vi "Table_CellValue_Tests.vi"(8 "error in":errorcluster) -> (0 "error out":errorcluster)   [LabVIEW 2016, in "DronaTest.lvlib"]
uses:
  DronaTest.lvlib
  APIs/Stimulus/ControlValue/SetValueAuto.vi
  APIs/Stimulus/ControlValue/Controls/Table/EditCellValue.vi
  APIs/Assert/AssertControlValue/Controls/Table/AssertCellValue.vi
  <vilib>/addons/_JKI Toolkits/Caraya/classes/Assert/Assert Error.vi
  APIs/Stimulus/ControlValue/Controls/Table/SetValue.vi
  <vilib>/addons/_JKI Toolkits/Caraya/classes/Test/Test.lvclass
  <vilib>/SLL Toolkit/SLL Debug/SLL Debug.lvlib
  Drona.lvlib
  <vilib>/addons/_JKI Toolkits/Caraya/classes/Assert/Assert.lvclass
  APIs/Stimulus/ControlValue/Controls/Table/StimulusTable.lvlib
  APIs/Assert/AssertControlValue/Controls/Table/AssertTable.lvlib
  APIs/Stimulus/ControlValue/ControlValue.lvlib
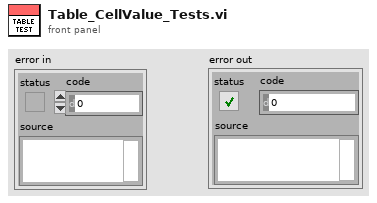
[diagram p1: front panel]
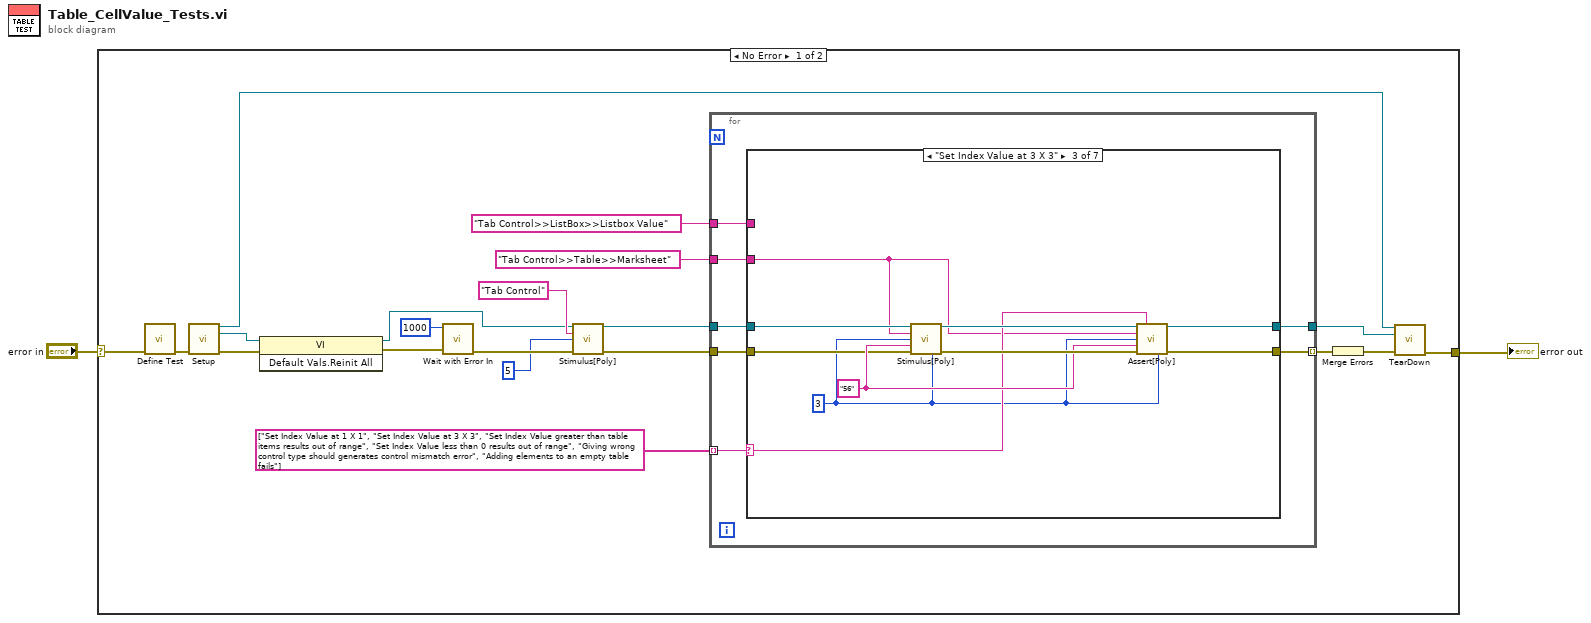
[diagram p0: block diagram]
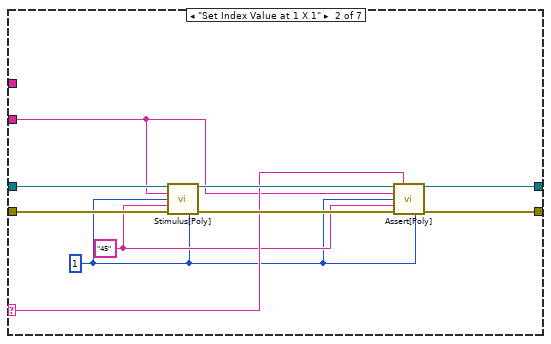
[diagram p3: hidden frame]
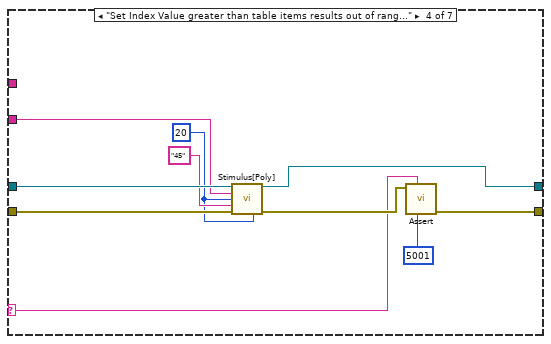
[diagram p4: hidden frame]
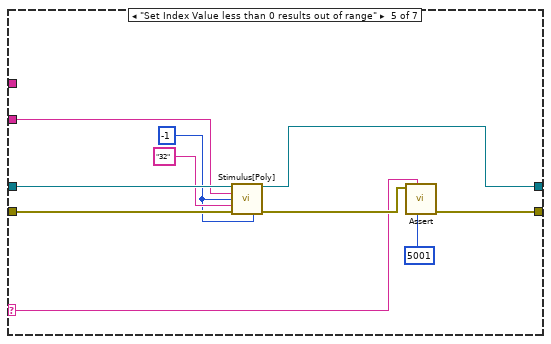
[diagram p5: hidden frame]
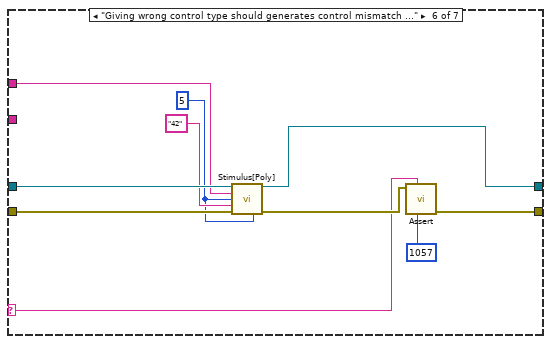
[diagram p6: hidden frame]
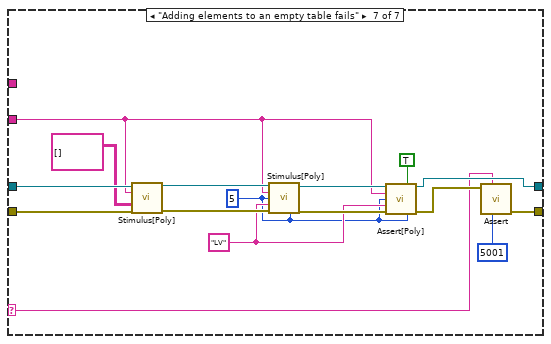
[diagram p7: hidden frame]
diagram:
  n1 = case shown="No Error" "error in" {
    selector: "error in" -> [w22 w98]
    tunnel: [w8 w98] -> w1
    frame No Error {
      n2 = call <vilib>:"Define Test.vi"("error in (no error)"=w22) -> ("error out"=w12:errorcluster)  [unwired: 9 in, 1 out]
      n3 = call "Setup.vi"("error in"=w12) -> ("Application Ref"=w10:refnum<vi>, "VI out"=w4:refnum<vi>, "error out"=w6:errorcluster)  [unwired: 12 in]
      n4 = invoke class="VI" method="Default Vals.Reinit All"(reference=w4, error in=w6) -> (reference out=w3:refnum<vi>, error out=w5:errorcluster)  [unwired: 1 in, 1 out]
      n5 = call <vilib>:"Wait with Error In.vi"("error in (no error)"=w5, "milliseconds to wait"=u32 1000) -> ("error out"=w20:errorcluster)  [unwired: 9 in]
      n6 = call-poly "Stimulus[Poly].vi"("VI Reference In"=w3, "Control Path"="Tab Control", "Value (Signaling)"=5, "error in"=w20) -> ("VI Reference Out"=w16:refnum<vi>, "error out"=w19:errorcluster)  [unwired: 10 in]
      n7 = for {
        tunnel: w16 -> [w28]
        tunnel: "Tab Control>>Table>>Marksheet" ("Control Path") -> [w27]
        tunnel: "Tab Control>>ListBox>>Listbox Value" ("Control Path") -> [w26]
        tunnel: string[] ["Set Index Value at 1 X 1", "Set Index Value at 3 X 3", "Set Index Value greater than table items results out of range", "Set Index Value less than 0 results out of range", "Giving wrong control type should generates control mismatch error", "Adding elements to an empty table fails"] -> [w24] mode=indexing
        tunnel: [w23] -> w9
        tunnel: w19 -> [w29]
        tunnel: [w25] -> w13 mode=indexing
        n8 = case shown="\"Set Index Value at 3 X 3\"" w24 {
          selector: w24 -> [_ w35 w44 w56 w66 w77 w84]
          tunnel: w29 -> [w31 w41 w47 w61 w71 w81 w97]
          tunnel: w28 -> [w30 w40 w48 w60 w70 w80 w95]
          tunnel: w27 -> [_ w33 w43 w59 w69 _ w90]
          tunnel: w26 -> [_ _ _ _ _ w74 _]
          tunnel: [w31 w37 w45 w57 w67 w78 w85] -> w25
          tunnel: [w30 w36 w46 w54 w64 w75 w87] -> w23
          frame Default {
          }
          frame "Set Index Value at 1 X 1" {
            w34 = "45" ("Value")
            w32 = 1 ("Item Index")
            n9 = call-poly "Stimulus[Poly].vi"("VI Reference In"=w40, "Control Path"=w33, "Row Index"=w32, "Value"=w34, "Error In"=w41, "Column Index"=w32) -> ("VI Reference Out"=w38:refnum<vi>, "Error Out"=w39:errorcluster)  [unwired: 8 in]
            n10 = call-poly "Assert[Poly].vi"("VI Reference In"=w38, "Test Label"=w35, "Control Path"=w33, "Row Index"=w32, "Item Value"=w34, "Error In"=w39, "Column Index"=w32) -> ("VI Reference Out"=w36:refnum<vi>, "Error Out"=w37:errorcluster)  [unwired: 6 in, 1 out]
          }
          frame "Set Index Value at 3 X 3" {
            w49 = "56" ("Value")
            w42 = 3 ("Item Index")
            n11 = call-poly "Stimulus[Poly].vi"("VI Reference In"=w48, "Control Path"=w43, "Row Index"=w42, "Value"=w49, "Error In"=w47, "Column Index"=w42) -> ("VI Reference Out"=w50:refnum<vi>, "Error Out"=w51:errorcluster)  [unwired: 8 in]
            n12 = call-poly "Assert[Poly].vi"("VI Reference In"=w50, "Test Label"=w44, "Control Path"=w43, "Row Index"=w42, "Item Value"=w49, "Error In"=w51, "Column Index"=w42) -> ("VI Reference Out"=w46:refnum<vi>, "Error Out"=w45:errorcluster)  [unwired: 6 in, 1 out]
          }
          frame "Set Index Value greater than table items results out of range" {
            w52 = 20 ("Item Index")
            n13 = call-poly "Stimulus[Poly].vi"("VI Reference In"=w60, "Control Path"=w59, "Row Index"=w52, "Value"="45", "Error In"=w61, "Column Index"=w52) -> ("VI Reference Out"=w54:refnum<vi>, "Error Out"=w58:errorcluster)  [unwired: 8 in]
            n14 = call-poly <vilib>:"Assert.vi"("error code (1)"=5001, "Label"=w56, "Error?"=w58) -> ("error out"=w57:errorcluster)  [unwired: 7 in, 1 out]
          }
          frame "Set Index Value less than 0 results out of range" {
            w62 = -1 ("Item Index")
            n15 = call-poly "Stimulus[Poly].vi"("VI Reference In"=w70, "Control Path"=w69, "Row Index"=w62, "Value"="32", "Error In"=w71, "Column Index"=w62) -> ("VI Reference Out"=w64:refnum<vi>, "Error Out"=w68:errorcluster)  [unwired: 8 in]
            n16 = call-poly <vilib>:"Assert.vi"("error code (1)"=5001, "Label"=w66, "Error?"=w68) -> ("error out"=w67:errorcluster)  [unwired: 7 in, 1 out]
          }
          frame "Giving wrong control type should generates control mismatch error" {
            w72 = 5 ("Item Index")
            n17 = call-poly "Stimulus[Poly].vi"("VI Reference In"=w80, "Control Path"=w74, "Row Index"=w72, "Value"="42", "Error In"=w81, "Column Index"=w72) -> ("VI Reference Out"=w75:refnum<vi>, "Error Out"=w79:errorcluster)  [unwired: 8 in]
            n18 = call-poly <vilib>:"Assert.vi"("error code (1)"=1057, "Label"=w77, "Error?"=w79) -> ("error out"=w78:errorcluster)  [unwired: 7 in, 1 out]
          }
          frame "Adding elements to an empty table fails" {
            w89 = "LV" ("Value")
            w82 = 5 ("Row Index")
            n19 = call-poly "Stimulus[Poly].vi"("VI Reference In"=w95, "Control Path"=w90, "Value"=string[][] [], "Error In"=w97) -> ("VI Reference Out"=w93:refnum<vi>, "Error Out"=w96:errorcluster)  [unwired: 10 in]
            n20 = call-poly "Stimulus[Poly].vi"("VI Reference In"=w93, "Control Path"=w90, "Row Index"=w82, "Value"=w89, "Error In"=w96, "Column Index"=w82) -> ("VI Reference Out"=w91:refnum<vi>, "Error Out"=w92:errorcluster)  [unwired: 8 in]
            n21 = call-poly "Assert[Poly].vi"("VI Reference In"=w91, "Assert Only? (F)"=TRUE, "Control Path"=w90, "Row Index"=w82, "Item Value"=w89, "Error In"=w92, "Column Index"=w82) -> ("VI Reference Out"=w87:refnum<vi>, "Error Out"=w86:errorcluster)  [unwired: 6 in, 1 out]
            n22 = call-poly <vilib>:"Assert.vi"("error code (1)"=5001, "Label"=w84, "Error?"=w86) -> ("error out"=w85:errorcluster)  [unwired: 7 in, 1 out]
          }
        }
      }
      n23 = Merge Errors(w13) -> (w11:errorcluster)
      n24 = call "TearDown.vi"("Application Ref"=w10, "VI in"=w9, "error in (no error)"=w11) -> ("error out"=w8:errorcluster)  [unwired: 12 in]
    }
    frame Error {
    }
  }
  "error out" <- w1
